vi "Performance Values.vi"(8 "error in (no error)":errorcluster, 11 "Linux System SAL in":refnum<class "Linux System SAL.lvclass">) -> (0 "error out":errorcluster, 2 "Performance Values":T1)   [LabVIEW 2020, in "Volatus.lvlib" / "Linux System SAL.lvclass"]
uses:
  Linux System SAL.lvclass
  System SAL/Performance Values.ctl
  Linux System SAL.lvclass/Linux System SAL.ctl
  System SAL/System SAL.lvclass
  <resource>/objmgr/nisysapi.rc
  <vilib>/Analysis/NI_AALBase.lvlib
  <vilib>/Analysis/baseanly.llb/Mean (DBL).vi
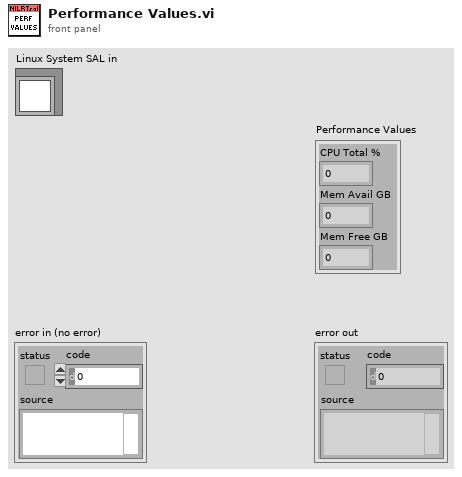
[diagram p1: front panel]
types:
  T1 = typedef "Volatus.lvlib/System SAL.lvclass/Performance Values.ctl" = cluster{"CPU Total %":dbl, "Mem Avail GB":dbl, "Mem Free GB":dbl}
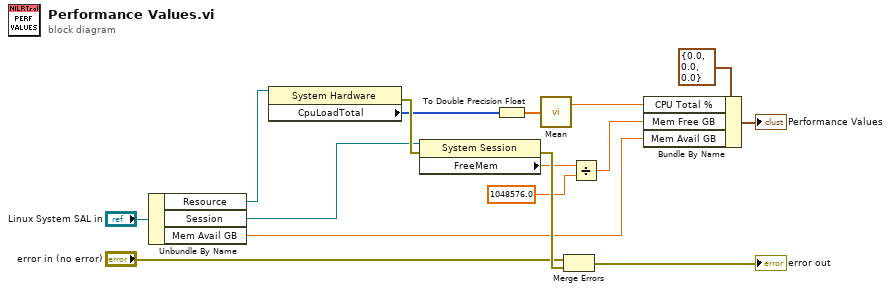
[diagram p0: block diagram]
diagram:
  n1 = Unbundle By Name("Linux System SAL in") -> ("Resource"=w13:refnum<k20>, "Session"=w9:refnum<k21>, "Mem Avail GB"=w8:dbl)
  n2 = property class="System Hardware"(reference=w13) -> (error out=w15:errorcluster, "CpuLoadTotal"=w12:u32[])  [unwired: 1 in, 1 out]
  n3 = property class="System Session"(reference=w9, error in=w15) -> (error out=w16:errorcluster, "FreeMem"=w7:dbl)  [unwired: 1 out]
  n4 = To Double Precision Float(number=w12) -> (double precision float=w11:dbl[])
  n5 = call-poly <vilib>:"Mean.vi"("X"=w11) -> ("mean"=w10:dbl)  [unwired: 1 out]
  n6 = Merge Errors("error in (no error)", w16) -> (→"error out":errorcluster)
  n7 = Divide(x=w7, y=1048576.0) -> (x/y=w5:dbl)
  n8 = Bundle By Name(cluster=T1 {"CPU Total %"=0.0, "Mem Avail GB"=0.0, "Mem Free GB"=0.0} ("Performance Values"), "CPU Total %"=w10, "Mem Free GB"=w5, "Mem Avail GB"=w8) -> (→"Performance Values":T1)
